vi "gdi32 CreateRectRgn.vi"(0 "x1":i32, 5 "y1":i32, 7 "x2":i32, 9 "y2":i32, 11 "error in":errorcluster) -> (4 "HRGN":u64, 15 "error out":errorcluster)   [LabVIEW 2020, in "RemoteVI.lvlib"]
doc: "Creates the rectangular region (x1, y1)-(x2, y2) through gdi32.dll CreateRectRgn (stdcall, called in any thread). 0, 0, 0, 0 gives an EMPTY region - given to a window with user32 SetWindowRgn.vi it makes the window invisible on screen while it stays open, functional and capturable with PrintWindow (measured on a LabVIEW menu). A region handed to SetWindowRgn belongs to the system afterwards; any other region must be deleted with gdi32 DeleteObject.vi. When error in carries an error the DLL is not called. Generated by scripts\\Build Win32 Wrappers.vi - do not edit by hand, rebuild it."
uses:
  RemoteVI.lvlib
  gdi32.dll
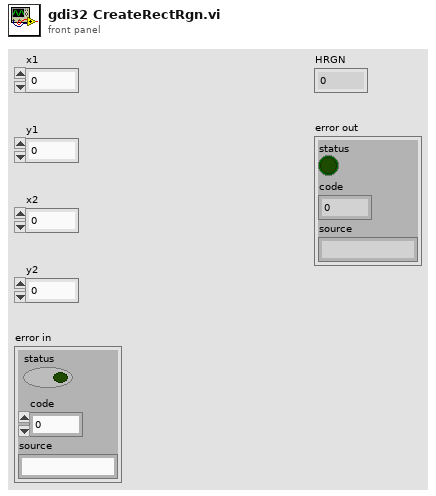
[diagram p1: front panel]
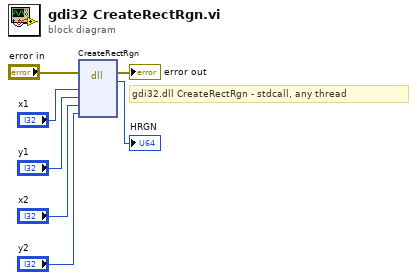
[diagram p0: block diagram]
diagram:
  # "gdi32.dll CreateRectRgn - stdcall, any thread"
  n1 = dll-call lib="gdi32.dll" fn="CreateRectRgn"(error in="error in", "x1"="x1", "y1"="y1", "x2"="x2", "y2"="y2") -> (error out=→"error out":errorcluster, →"HRGN":u64)  [unwired: 6 in, 1 out]
